vi "Completer_un_tableau.vi"(2 "Remplir jusqu'à":u32, 3 "Tableau en entrée":dbl[](array[numeric])) -> (0 "Afficher ?":bool, 1 "Tableau en sortie":dbl[](array[numeric]))   [LabVIEW 2022 SP3]
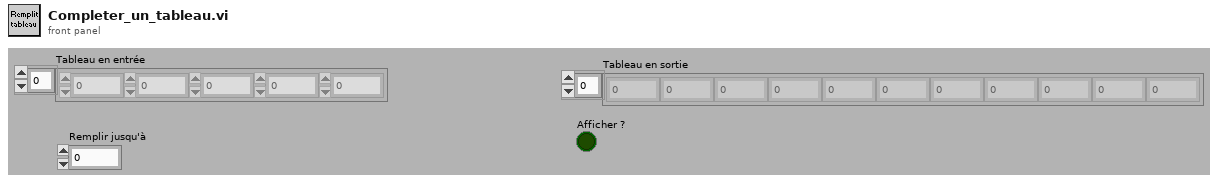
[diagram p1: front panel]
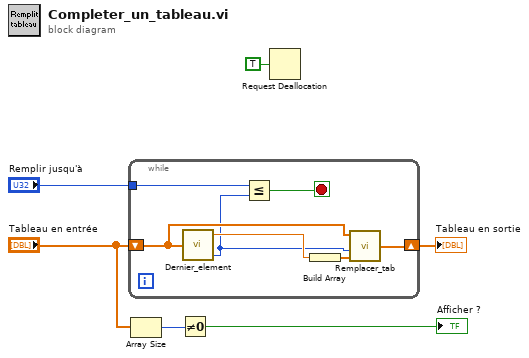
[diagram p0: block diagram]
diagram:
  n1 = while {
    tunnel: "Remplir jusqu'à" -> [w13]
    shift-right: [w9] -> w5
    shift-left: "Tableau en entrée" -> [w8]
    stop <- w12 stop-if-true
    n2 = call "Dernier_element.vi"("Tableau en entrée"=w8) -> ("Dernier élément"=w10:dbl, "Taille/Indice N+1"=w7:i32)  [unwired: 1 out]
    n3 = Less Or Equal?(x=w13, y=w7) -> (x <= y?=w12:bool)
    n4 = Build Array(w10) -> (w11:dbl[])
    n5 = call "Remplacer_tab.vi"("Nouvel élément/sous tableau"=w11, "A partir de"=w7, "Tableau"=w8) -> ("Tableau inséré/remplacé"=w9:dbl[])  [unwired: 1 in]
  }
  "Tableau en sortie" <- w5
  n6 = Array Size(array="Tableau en entrée") -> (size(s)=w3:i32)
  n7 = Not Equal To 0?(x=w3) -> (x != 0?=→"Afficher ?":bool)
  n8 = Request Deallocation(TRUE ("flag")) -> ()
